vi "GetAllPropertyName.vi"(10 "NewPropertyName":string, 11 "Data":T1) -> (3 "Duplicated Name?":bool)   [LabVIEW 2017]
uses:
  Ctrl/Data.ctl
  Ctrl/Caps.ctl
  Ctrl/Property.ctl
  Ctrl/PhysicalChannel.ctl
  Ctrl/Register.ctl
  Ctrl/Bitfield.ctl
  Ctrl/Scale.ctl
  Ctrl/ScaleType.ctl
  Ctrl/Enum.ctl
  Ctrl/EnumValue.ctl
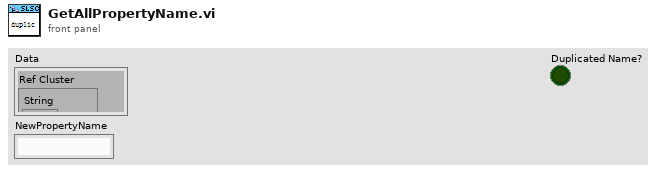
[diagram p1: front panel]
types:
  T1 = typedef "Data.ctl" = cluster{"Ref Cluster":cluster{"String":refnum<vi>, "U8":refnum<vi>, "I8":refnum<vi>, "U32":refnum<vi>, "I32":refnum<vi>, "U64":refnum<vi>, "I64":refnum<vi>, "Ring":refnum<vi>, "DBL":refnum<vi>, "Add":refnum<vi>, "Remove":refnum<vi>, "Property tree":refnum<vi>, "confirm":refnum<vi>}, "JSON Text":string, "Original JSON Text":string, "Caps":T2, "SLSC Output Tree":cluster{"Left Cell String":string, "Child Text":string[], "Child Tag":string, "Item Indent":i32, "Child Only?":bool, "Glyph Index":i32, "offline value":variant}[], "Ref Index and Control Type":cluster{"index":i32, "Datatype":string}, "Selected Type and name":cluster{"Selected Type":enum16{"Property", "Physical Channel", "Other"}, "Selected Property Name":string}, "Update whole Tree?":bool}
  T2 = typedef "Caps.ctl" = cluster{"properties":T3[], "physical channels":T4[], "registers":T5[], "scales":T7[], "enums":T9[], "productName":string}
  T3 = typedef "Property.ctl" = cluster{"name":string, "bitfield":string, "value":variant, "dataType":string, "min":variant, "max":variant, "scale":string, "access":string}
  T4 = typedef "PhysicalChannel.ctl" = cluster{"name":string, "properties":T3[]}
  T5 = typedef "Register.ctl" = cluster{"name":string, "address":i32, "size":i32, "bitfields":T6[], "initialValue":variant, "connectedProperties":string[]}
  T6 = typedef "Bitfield.ctl" = cluster{"name":string, "offset":i32, "size":i32, "signed":bool}
  T7 = typedef "Scale.ctl" = cluster{"name":string, "type":T8, "params":variant}
  T8 = typedef "ScaleType.ctl" = enum16{"NoScale", "Table", "Polynomial", "Linear"}
  T9 = typedef "Enum.ctl" = cluster{"name":string, "values":T10[]}
  T10 = typedef "EnumValue.ctl" = cluster{"name":string, "value":i32}
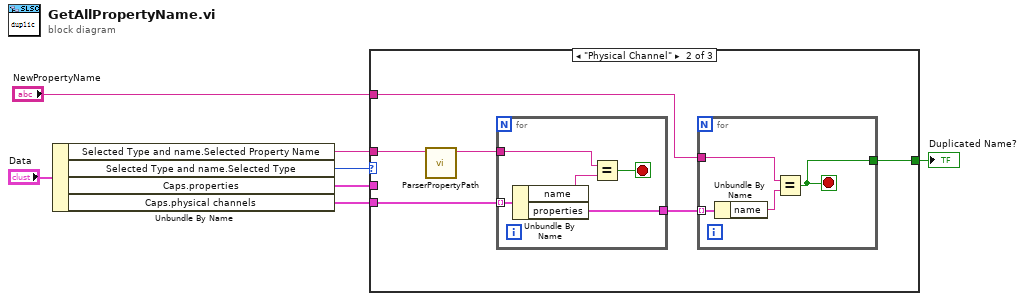
[diagram p0: block diagram]
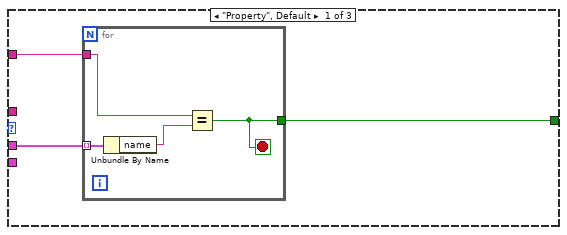
[diagram p2: hidden frame]
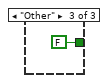
[diagram p3: hidden frame]
diagram:
  n1 = Unbundle By Name("Data") -> ("Selected Type and name.Selected Property Name"=w2:string, "Selected Type and name.Selected Type"=w6:enum16{"Property", "Physical Channel", "Other"}, "Caps.properties"=w5:T3[], "Caps.physical channels"=w4:T4[])
  n2 = case shown="\"Physical Channel\"" w6 {
    tunnel: w5 -> [w10 _ _]
    tunnel: w4 -> [_ w18 _]
    tunnel: "NewPropertyName" -> [w9 w16 _]
    tunnel: [w8 w15 FALSE] -> w1
    tunnel: w2 -> [_ w20 _]
    frame "Property", Default {
      n3 = for {
        tunnel: w10 -> [w14] mode=indexing
        tunnel: w9 -> [w12]
        tunnel: [w11] -> w8
        stop <- w11 stop-if-true
        n4 = Unbundle By Name(w14) -> ("name"=w13:string)
        n5 = Equal?(x=w12, y=w13) -> (x = y?=w11:bool)
      }
    }
    frame "Physical Channel" {
      n6 = call "ParserPropertyPath.vi"("Seleted Item Name"=w20) -> ("Physical channel"=w19:string)  [unwired: 7 in, 1 out]
      n7 = for {
        tunnel: w19 -> [w28]
        tunnel: w18 -> [w29] mode=indexing
        tunnel: [w25] -> w17
        stop <- w26 stop-if-true
        n8 = Unbundle By Name(w29) -> ("name"=w27:string, "properties"=w25:T3[])
        n9 = Equal?(x=w28, y=w27) -> (x = y?=w26:bool)
      }
      n10 = for {
        tunnel: w17 -> [w24] mode=indexing
        tunnel: w16 -> [w22]
        tunnel: [w21] -> w15
        stop <- w21 stop-if-true
        n11 = Unbundle By Name(w24) -> ("name"=w23:string)
        n12 = Equal?(x=w22, y=w23) -> (x = y?=w21:bool)
      }
    }
    frame "Other" {
    }
  }
  "Duplicated Name?" <- w1
